vi "Cell Value to Numeric.vi"(11 "Cell Value":string) -> (1 "Unit":string, 3 "Numeric":dbl format="%#_6p")   [LabVIEW 2026, in "Digital Pattern Sequencer.lvclass"]
uses:
  Digital Pattern Sequencer.lvclass
  <vilib>/Utility/error.llb/Trim Whitespace One-Sided.vi
  <vilib>/regexp/Match Regular Expression.xnode
  Digital Pattern Sequencer.lvclass/Digital Pattern Sequencer.ctl
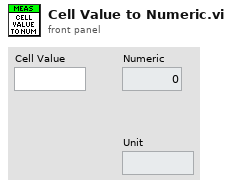
[diagram p1: front panel]
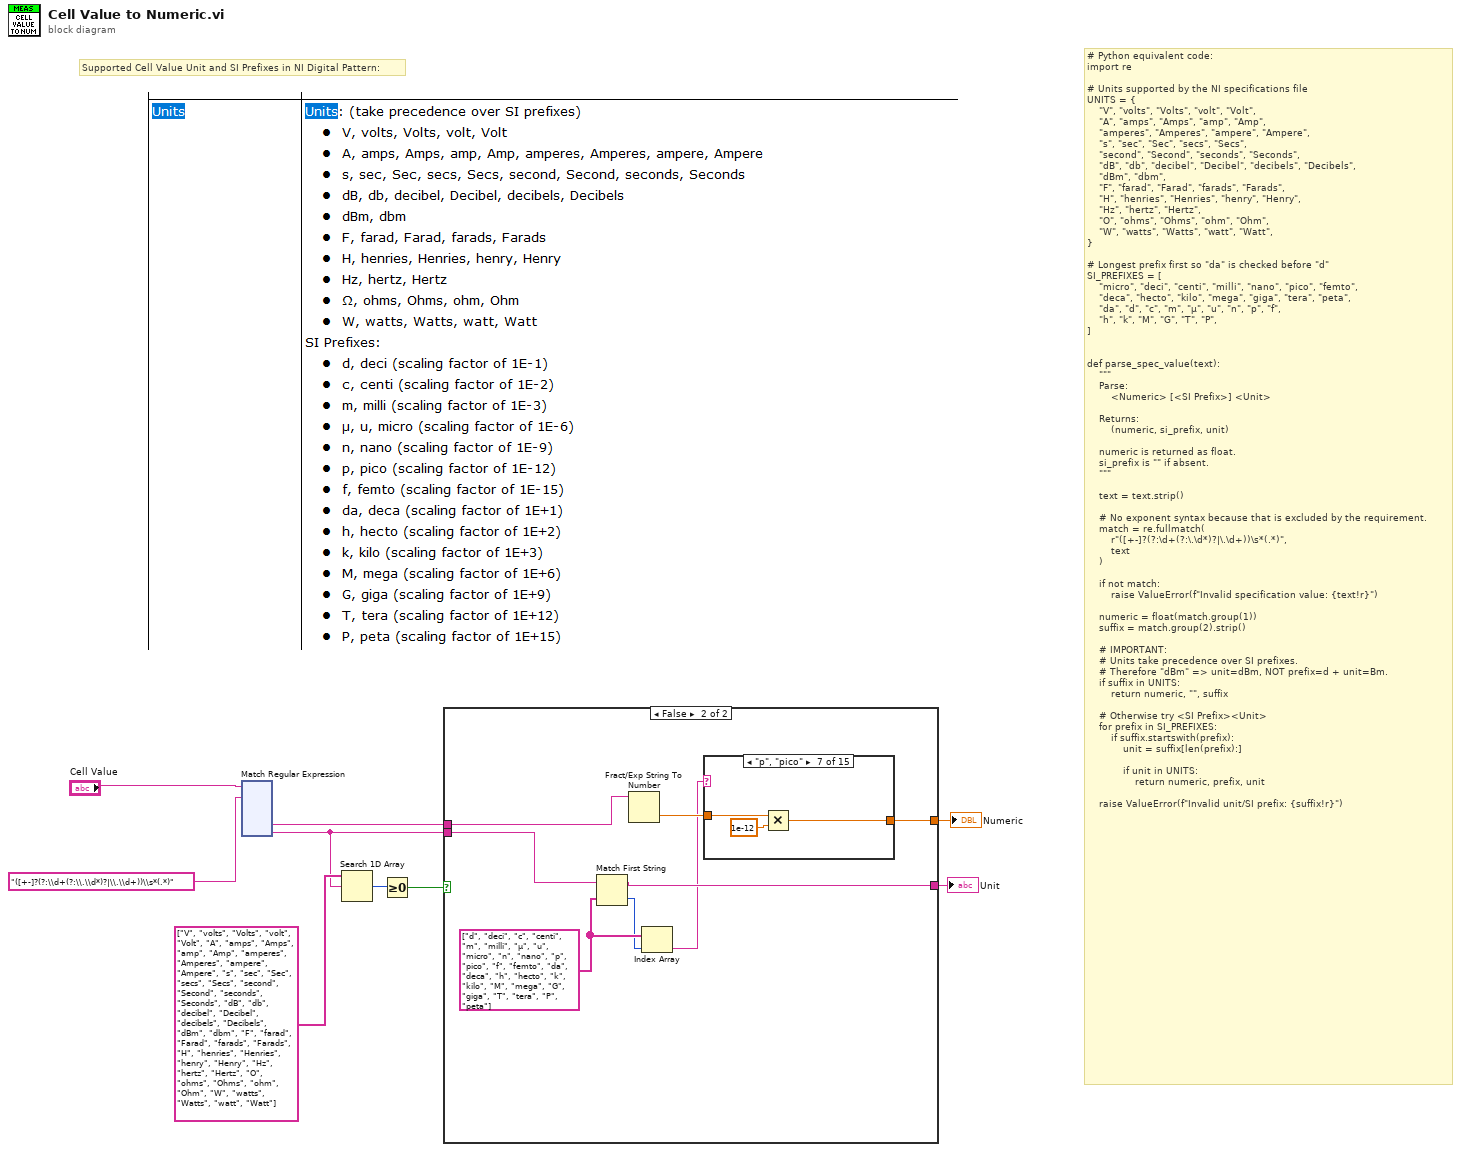
[diagram p0: block diagram]
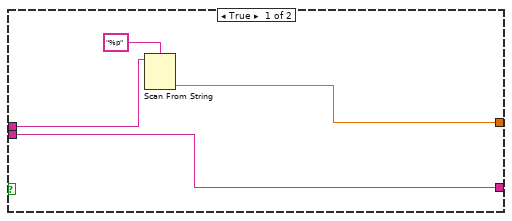
[diagram p2: hidden frame]
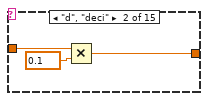
[diagram p4: hidden frame]
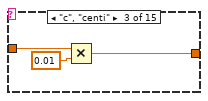
[diagram p5: hidden frame]
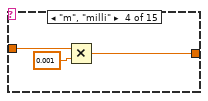
[diagram p6: hidden frame]
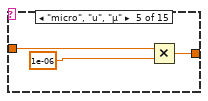
[diagram p7: hidden frame]
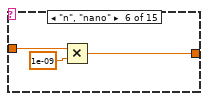
[diagram p8: hidden frame]
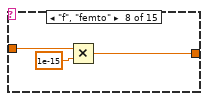
[diagram p9: hidden frame]
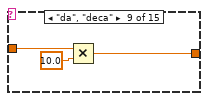
[diagram p10: hidden frame]
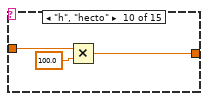
[diagram p11: hidden frame]
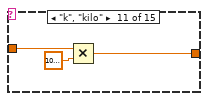
[diagram p12: hidden frame]
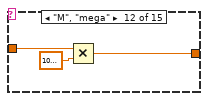
[diagram p13: hidden frame]
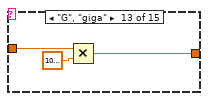
[diagram p14: hidden frame]
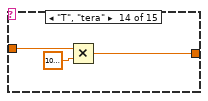
[diagram p15: hidden frame]
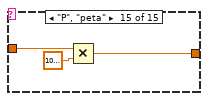
[diagram p16: hidden frame]
diagram:
  # "# Python equivalent code:\nimport re\n\n# Units supported by the NI specifications file\nUNITS = {\n    \"V\", \"volts\", \"Volts\", \"volt\", \"Volt\",\n    \"A\", \"amps\", \"Amps\", \"amp\", \"Amp\",\n    \"amperes\", \"Amperes\", \"ampere\", \"Ampere\",\n    \"s\", \"sec\", \"Sec\", \"secs\", \"Secs\",\n    \"second\", \"Second\", \"seconds\", \"Seconds\",\n    \"dB\", \"db\", \"decibel\", \"Decibel\", \"decibels\", \"Decibels\",\n    \"dBm\", \"dbm\",\n    \"F\", \"farad\", \"Farad\", \"farads\", \"Farads\",\n    \"H\", \"henries\", \"Henries\", \"henry\", \"Henry\",\n    \"Hz\", \"hertz\", \"Hertz\",\n    \"O\", \"ohms\", \"Ohms\", \"ohm\", \"Ohm\",\n    \"W\", \"watts\", \"Watts\", \"watt\", \"Watt\",\n}\n\n# Longest prefix first so \"da\" is checked before \"d\"\nSI_PREFIXES = [\n    \"micro\", \"deci\", \"centi\", \"milli\", \"nano\", \"pico\", \"femto\",\n    \"deca\", \"hecto\", \"kilo\", \"mega\", \"giga\", \"tera\", \"peta\",\n    \"da\", \"d\", \"c\", \"m\", \"µ\", \"u\", \"n\", \"p\", \"f\",\n    \"h\", \"k\", \"M\", \"G\", \"T\", \"P\",\n]\n\n\ndef parse_spec_value(text):\n    \"\"\"\n    Parse:\n        <Numeric> [<SI Prefix>] <Unit>\n\n    Returns:\n        (numeric, si_prefix, unit)\n\n    numeric is returned as float.\n    si_prefix is \"\" if absent.\n    \"\"\"\n\n    text = text.strip()\n\n    # No exponent syntax because that is excluded by the requirement.\n    match = re.fullmatch(\n        r\"([+-]?(?:\\d+(?:\\.\\d*)?|\\.\\d+))\\s*(.*)\",\n        text\n    )\n\n    if not match:\n        raise ValueError(f\"Invalid specification value: {text!r}\")\n\n    numeric = float(match.group(1))\n    suffix = match.group(2).strip()\n\n    # IMPORTANT:\n    # Units take precedence over SI prefixes.\n    # Therefore \"dBm\" => unit=dBm, NOT prefix=d + unit=Bm.\n    if suffix in UNITS:\n        return numeric, \"\", suffix\n\n    # Otherwise try <SI Prefix><Unit>\n    for prefix in SI_PREFIXES:\n        if suffix.startswith(prefix):\n            unit = suffix[len(prefix):]\n\n            if unit in UNITS:\n                return numeric, prefix, unit\n\n    raise ValueError(f\"Invalid unit/SI prefix: {suffix!r}\")"
  # "Supported Cell Value Unit and SI Prefixes in NI Digital Pattern:"
  n1 = xnode "Match Regular Expression"("input string"="Cell Value", "regular expression"="([+-]?(?:\\d+(?:\\.\\d*)?|\\.\\d+))\\s*(.*)") -> ("submatch 1"=w8:string, "submatch 2"=w5:string)  [unwired: 4 in, 5 out]
  n2 = Search 1D Array(1D array=string[] ["V", "volts", "Volts", "volt", "Volt", "A", "amps", "Amps", "amp", "Amp", "amperes", "Amperes", "ampere", "Ampere", "s", "sec", "Sec", "secs", "Secs", "second", "Second", "seconds", "Seconds", "dB", "db", "decibel", "Decibel", "decibels", "Decibels", "dBm", "dbm", "F", "farad", "Farad", "farads", "Farads", "H", "henries", "Henries", "henry", "Henry", "Hz", "hertz", "Hertz", "O", "ohms", "Ohms", "ohm", "Ohm", "W", "watts", "Watts", "watt", "Watt"], element=w5) -> (index of element=w4:i32)  [unwired: 1 in]
  n3 = Greater Or Equal To 0?(x=w4) -> (x >= 0?=w3:bool)
  n4 = case shown="False" w3 {
    tunnel: w8 -> [w11 w17]
    tunnel: [w13 w21] -> w7
    tunnel: w5 -> [w13 w20]
    tunnel: [w10 w14] -> w2
    frame True {
      n5 = Scan From String(format string="%p", input string=w11) -> (output 1=w10:dbl)  [unwired: 3 in, 3 out]
    }
    frame False {
      w19 = string[] ["d", "deci", "c", "centi", "m", "milli", "µ", "u", "micro", "n", "nano", "p", "pico", "f", "femto", "da", "deca", "h", "hecto", "k", "kilo", "M", "mega", "G", "giga", "T", "tera", "P", "peta"]
      n6 = Match First String(2:w19, 3:w20) -> (0:w18:i32, 1:w21:string)
      n7 = Fract/Exp String To Number(string=w17) -> (number=w16:dbl)  [unwired: 3 in, 1 out]
      n8 = Index Array(array=w19, index=w18) -> (element=w15:string)
      n9 = case shown="\"p\", \"pico\"" w15 {
        tunnel: w16 -> [w22 w25 w28 w31 w33 w36 w39 w42 w45 w48 w51 w54 w57 w60 w63]
        tunnel: [w22 w23 w26 w29 w32 w35 w38 w41 w44 w47 w50 w53 w56 w59 w62] -> w14
        frame Default {
        }
        frame "d", "deci" {
          n10 = Multiply(x=w25, y=0.1) -> (x*y=w23:dbl)
        }
        frame "c", "centi" {
          n11 = Multiply(x=w28, y=0.01) -> (x*y=w26:dbl)
        }
        frame "m", "milli" {
          n12 = Multiply(x=w31, y=0.001) -> (x*y=w29:dbl)
        }
        frame "micro", "u", "µ" {
          n13 = Multiply(x=w33, y=1e-06) -> (x*y=w32:dbl)
        }
        frame "n", "nano" {
          n14 = Multiply(x=w36, y=1e-09) -> (x*y=w35:dbl)
        }
        frame "p", "pico" {
          n15 = Multiply(x=w39, y=1e-12) -> (x*y=w38:dbl)
        }
        frame "f", "femto" {
          n16 = Multiply(x=w42, y=1e-15) -> (x*y=w41:dbl)
        }
        frame "da", "deca" {
          n17 = Multiply(x=w45, y=10.0) -> (x*y=w44:dbl)
        }
        frame "h", "hecto" {
          n18 = Multiply(x=w48, y=100.0) -> (x*y=w47:dbl)
        }
        frame "k", "kilo" {
          n19 = Multiply(x=w51, y=1000.0) -> (x*y=w50:dbl)
        }
        frame "M", "mega" {
          n20 = Multiply(x=w54, y=1000000.0) -> (x*y=w53:dbl)
        }
        frame "G", "giga" {
          n21 = Multiply(x=w57, y=1000000000.0) -> (x*y=w56:dbl)
        }
        frame "T", "tera" {
          n22 = Multiply(x=w60, y=1000000000000.0) -> (x*y=w59:dbl)
        }
        frame "P", "peta" {
          n23 = Multiply(x=w63, y=1000000000000000.0) -> (x*y=w62:dbl)
        }
      }
    }
  }
  "Unit" <- w7
  "Numeric" <- w2
